vi "Calc Texel Starting Conditions.vi"(10 "Texture":T6, 11 "Sorted Triangle":T1={"Top Vertex"={"Position"={"x"=0.0, "y"=0.0, "z"=0.0}, "UV"={"u"=0.0, "v"=0.0}, "Colour"=12517256}, "Mid Vertex"={"Position"={"x"=0.0, "y"=0.0, "z"=0.0}, "UV"={"u"=0.0, "v"=0.0}, "Colour"=12517256}, "Bottom Vertex"={"Position"={"x"=0.0, "y"=0.0, "z"=0.0}, "UV"={"u"=0.0, "v"=0.0}, "Colour"=12517256}, "Alpha"=0.0, "Alpha Blending Enabled"=FALSE, "Colour"=0, "Material"={"Diffuse Colour"=0, "Texture"={"Pixels"=refnum, "Size"={"Width"=0, "Height"=0}}}} {"Bottom Vertex"."UV"."v" min=0 max=1 step=0.1; "Bottom Vertex"."UV"."u" min=0 max=1 step=0.1; "Mid Vertex"."UV"."v" min=0 max=1 step=0.1; "Mid Vertex"."UV"."u" min=0 max=1 step=0.1; "Top Vertex"."UV"."v" min=0 max=1 step=0.1; "Top Vertex"."UV"."u" min=0 max=1 step=0.1}) -> (3 "Step Deltas (Texels Per Step)":T8)   [LabVIEW 2020, in "Raster.lvlib"]
uses:
  Raster.lvlib
  Texel Step Deltas.ctl
  Point 2D (SGL).ctl
  UV.ctl
  Rectangle Dimensions.ctl
  Texture.ctl
  3D/Vector 3D.ctl
  3D/3D.lvlib
  3D/Vertex.ctl
  3D/Triangle (Sorted).ctl
  3D/Material.ctl
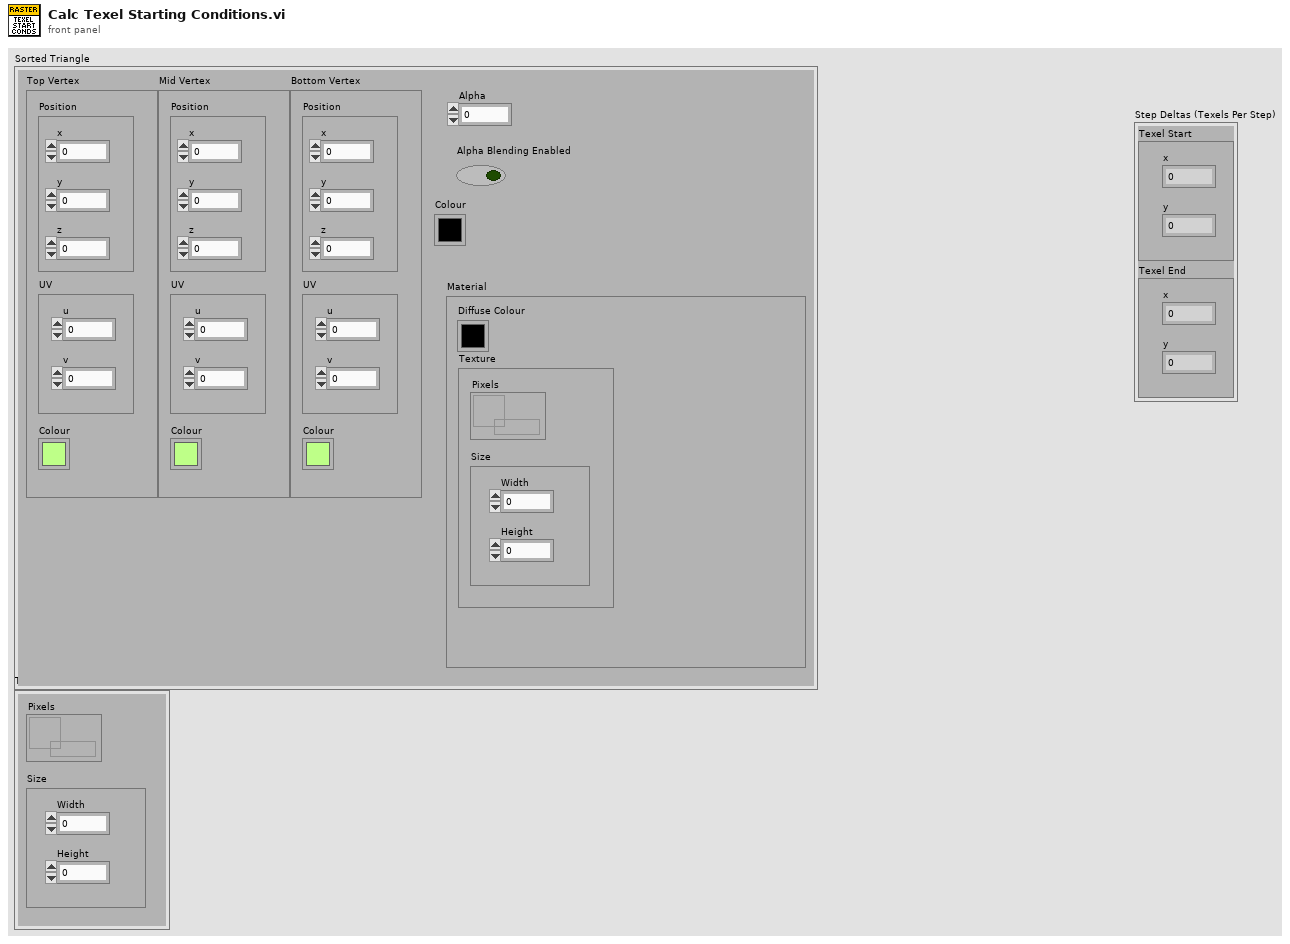
[diagram p1: front panel]
types:
  T1 = typedef "3D.lvlib/Triangle (Sorted).ctl" = cluster{"Top Vertex":T2, "Mid Vertex":T2, "Bottom Vertex":T2, "Alpha":dbl, "Alpha Blending Enabled":bool, "Colour":u32, "Material":T5}
  T2 = typedef "3D.lvlib/Vertex.ctl" = cluster{"Position":T3, "UV":T4, "Colour":u32}
  T3 = typedef "3D.lvlib/Vector 3D.ctl" = cluster{"x":sgl, "y":sgl, "z":sgl}
  T4 = typedef "Raster.lvlib/UV.ctl" = cluster{"u":sgl, "v":sgl}
  T5 = typedef "3D.lvlib/Material.ctl" = cluster{"Diffuse Colour":u32, "Texture":T6}
  T6 = typedef "Raster.lvlib/Texture.ctl" = cluster{"Pixels":refnum<data-value>, "Size":T7}
  T7 = typedef "Raster.lvlib/Rectangle Dimensions.ctl" = cluster{"Width":u32, "Height":u32}
  T8 = typedef "Raster.lvlib/Texel Step Deltas.ctl" = cluster{"Texel Start":T9, "Texel End":T9}
  T9 = typedef "Raster.lvlib/Point 2D (SGL).ctl" = cluster{"x":sgl, "y":sgl}
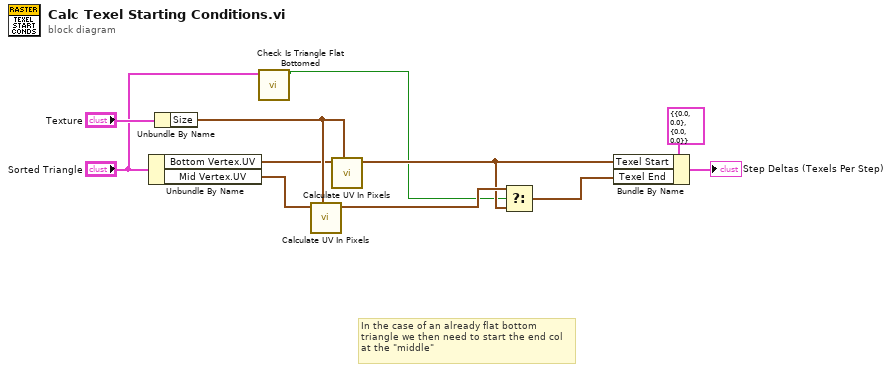
[diagram p0: block diagram]
diagram:
  # "In the case of an already flat bottom triangle we then need to start the end col at the \"middle\""
  n1 = Unbundle By Name("Sorted Triangle") -> ("Bottom Vertex.UV"=w4:T4, "Mid Vertex.UV"=w3:T4)
  n2 = Unbundle By Name("Texture") -> ("Size"=w5:T7)
  n3 = call "Check Is Triangle Flat Bottomed.vi"("Sorted Triangle"="Sorted Triangle") -> ("Flat Bottom Triangle"=w1:bool)  [unwired: 10 in]
  n4 = call "Calculate UV In Pixels.vi"("Texture Dimensions"=w5, "UV"=w3) -> ("Pixels"=w8:T9)  [unwired: 9 in]
  n5 = call "Calculate UV In Pixels.vi"("Texture Dimensions"=w5, "UV"=w4) -> ("Pixels"=w7:T9)  [unwired: 9 in]
  n6 = Select(t=w8, s=w1, f=w7) -> (s? t:f=w11:T9)
  n7 = Bundle By Name(cluster=T8 {"Texel Start"={"x"=0.0, "y"=0.0}, "Texel End"={"x"=0.0, "y"=0.0}} ("Step Deltas (Texels Per Step)"), "Texel Start"=w7, "Texel End"=w11) -> (→"Step Deltas (Texels Per Step)":T8)
